vi "test - Clear CSM Queue.vi"(8 "error in (no error)":errorcluster, 11 "TestCase in":refnum<class "testcase-Basic-Function.lvclass">) -> (0 "error out":errorcluster, 3 "TestCase out":refnum<class "testcase-Basic-Function.lvclass">)   [LabVIEW 2017, in "testcase-Basic-Function.lvclass"]
uses:
  testcase-Basic-Function.lvclass
  src/user.lib/_NEVSTOP/Communicable State Machine(CSM)/_Support/CSMQ/_CSMOFGVOPER.ctl
  src/user.lib/_NEVSTOP/Communicable State Machine(CSM)/AdvanceAPI/CSM - Revert Arguments-Safe String.vi
  src/user.lib/_NEVSTOP/Communicable State Machine(CSM)/_Shared/Trim Single-line Text.vi
  src/user.lib/_NEVSTOP/Communicable State Machine(CSM)/AdvanceAPI/CSM - Make String Arguments Safe.vi
  src/user.lib/_NEVSTOP/Communicable State Machine(CSM)/AdvanceAPI/CSM - Break Down Multiple States String.vi
  src/user.lib/_NEVSTOP/Communicable State Machine(CSM)/AdvanceAPI/CSM - Compact Multiple States.vi
  src/user.lib/_NEVSTOP/Communicable State Machine(CSM)/AdvanceAPI/CSM - Keywords.vi
  <vilib>/addons/_JKI Toolkits/VI Tester/TestCase.llb/TestCase.lvclass
  src/user.lib/_NEVSTOP/Communicable State Machine(CSM)/Communicable State Machine.lvlib
  C:/Program Files (x86)/National Instruments/LabVIEW 2017/vi.lib/addons/_JKI Toolkits/VI Tester/TestCase.llb/TestCase.lvclass
panel:
  out "# pending insert":i32
  out "# pending remove":i32
  out "#Flushed":cluster{i32, i32}
  out "#elements in queue":i32
  out "error out 5":errorcluster
  out "error out 4":errorcluster
  out "error out 3":errorcluster
  out "error out 2":errorcluster
  out "error out 1":errorcluster
  out "State History":string
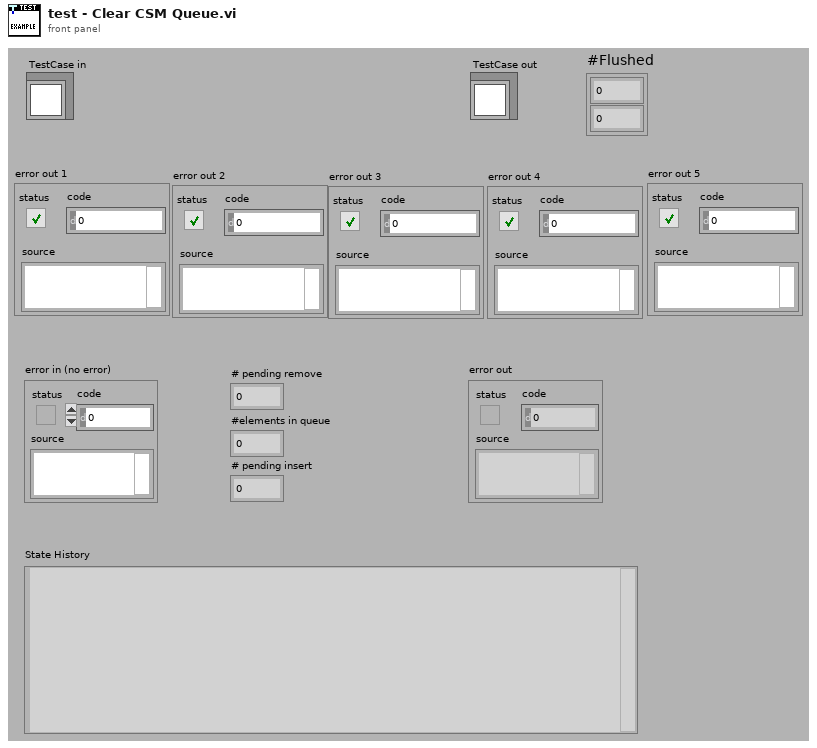
[diagram p1: front panel]
types:
  T1 = enum32{"Invalid", "Standard", "Closed", "Hidden", "Minimized", "Maximized"}
  T2 = enum32{"invalid app kind", "Development System", "Run Time System", "Student Edition", "Embedded LabVIEW", "Evaluation", "Custom"}
  T3 = typedef "Communicable State Machine.lvlib/_CSMOFGVOPER.ctl" = enum16{"Create If not Exist", "Get By Name", "List", "Check If Name Exists", "Release", "Module Status", "Create Status Event Handler", "Destroy Status Event Handler", "Clear Invalid Objs"}
  T4 = typedef "Communicable State Machine.lvlib/_CSM_Response Source Message.ctl" = cluster{"‘State":string, "’Arguments":string, "’Error":errorcluster}
  T5 = cluster{"Current VI Reference":refnum<vi>, "Close Panel on Exit?":bool}
  T6 = cluster{"Core":cluster{"Current VI Reference":refnum<vi>, "Close Panel on Exit?":bool}, "Your Boolean data":bool, "Your string data":string}
  T7 = typedef "Communicable State Machine.lvlib/_CSMObj.ctl" = cluster{"info":T8, "Refs":T10}
  T8 = typedef "Communicable State Machine.lvlib/_CSMObj-Info.ctl" = cluster{"Module Name":string, "Requested Name":string, "Group Name":string, "Mode":T9, "Allowed Messages":string[]}
  T9 = typedef "Communicable State Machine.lvlib/_CSM_MODE.ctl" = enum16{"Not Exist", "Stand Alone", "CSM", "Worker", "Worker Agent", "Chain Node", "Chain"}
  T10 = typedef "Communicable State Machine.lvlib/_CSMObj-Refs.ctl" = cluster{"WatchDogQ":refnum<queue>, "CSMDataDVR":refnum<data-value>, "Queue":T11, "GroupDataDVR":refnum<data-value>, "TagMap":refnum<data-value>, "ExitEvent":refnum<user-event>, "NewStateEvent":refnum<user-event>, "StatusEvent":refnum<user-event>, "InterruptEvent":refnum<user-event>}
  T11 = typedef "Communicable State Machine.lvlib/Priority Queue.ctl" = cluster{"HPriorityQ":refnum<queue>, "LowPriorityQ":refnum<queue>}
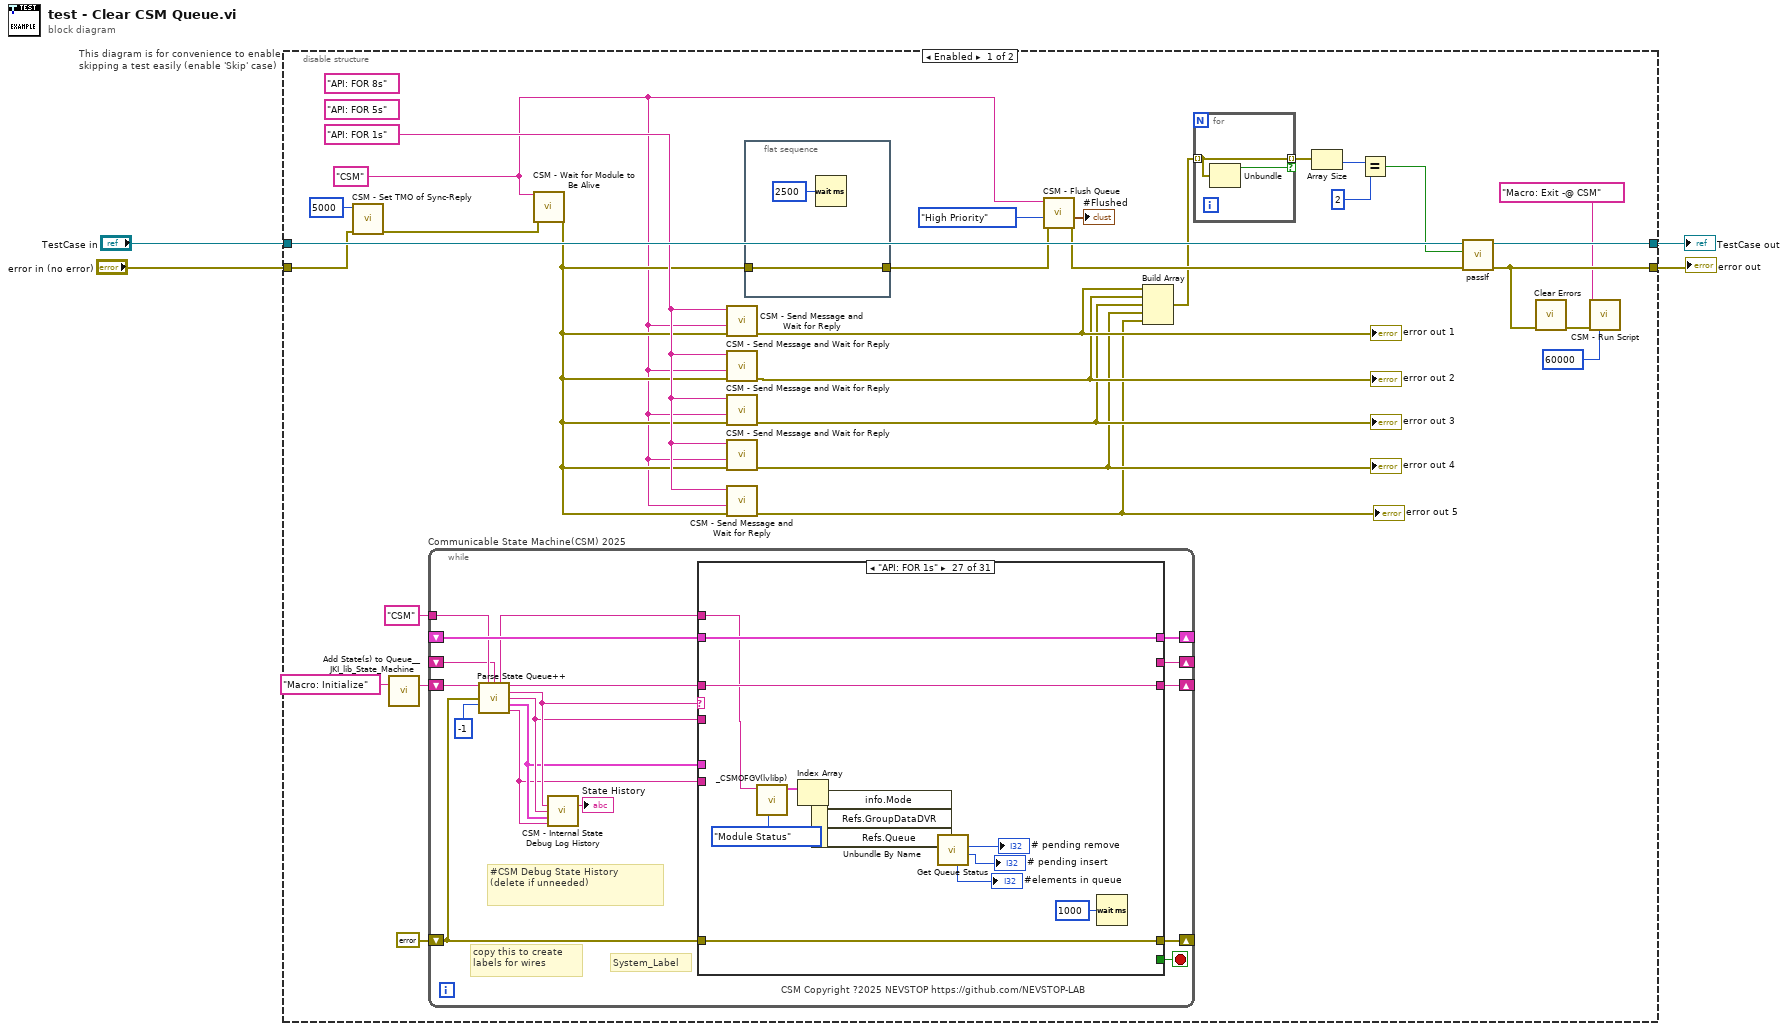
[diagram p0: block diagram]
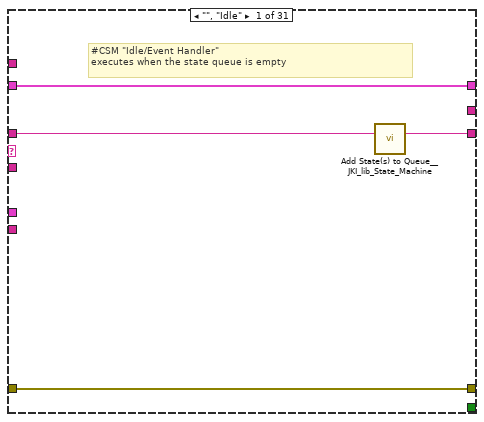
[diagram p2: hidden frame]
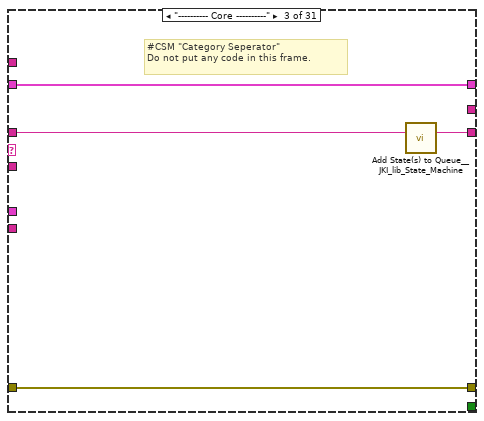
[diagram p4: hidden frame]
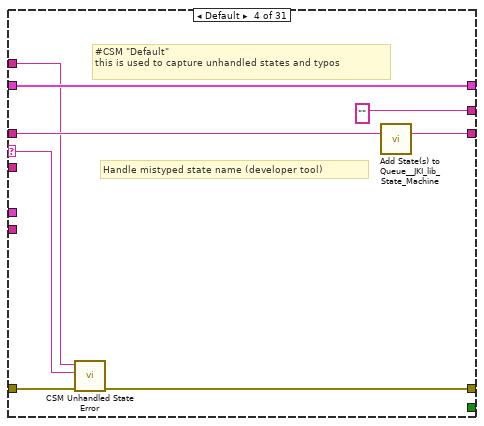
[diagram p5: hidden frame]
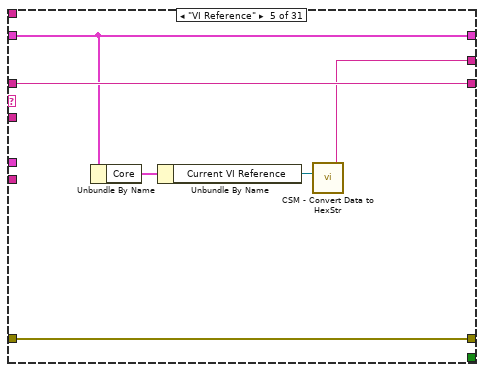
[diagram p6: hidden frame]
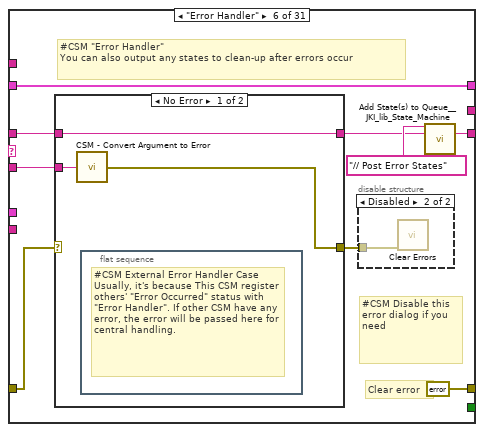
[diagram p7: hidden frame]
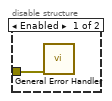
[diagram p8: hidden frame]
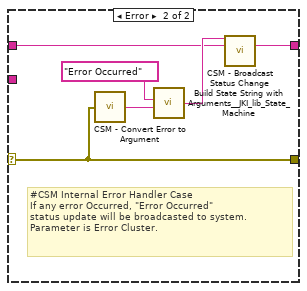
[diagram p9: hidden frame]
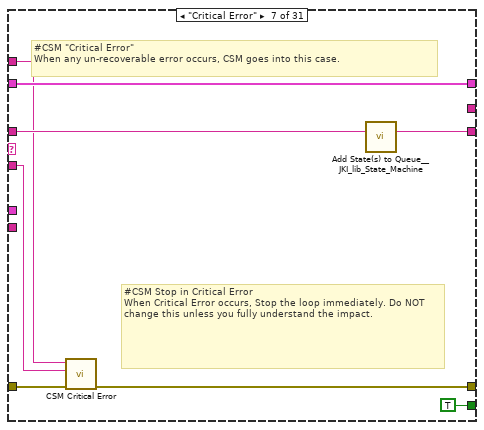
[diagram p10: hidden frame]
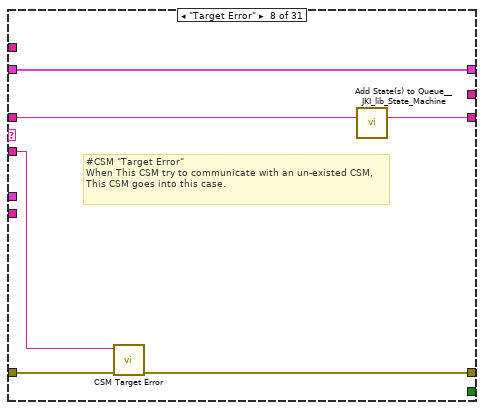
[diagram p11: hidden frame]
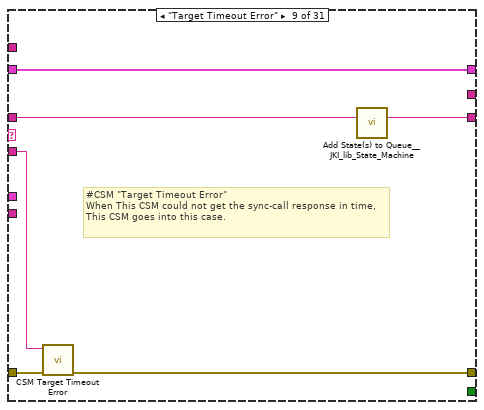
[diagram p12: hidden frame]
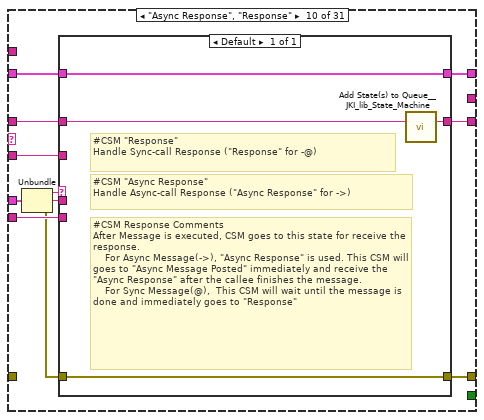
[diagram p13: hidden frame]
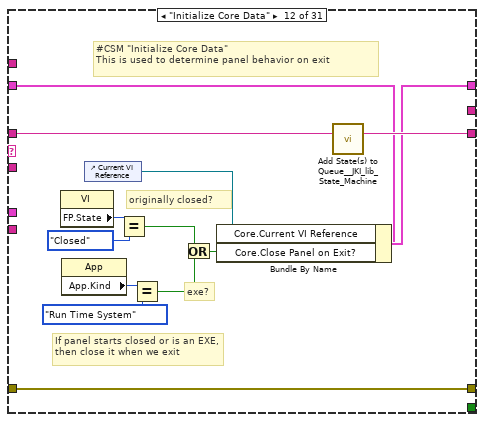
[diagram p15: hidden frame]
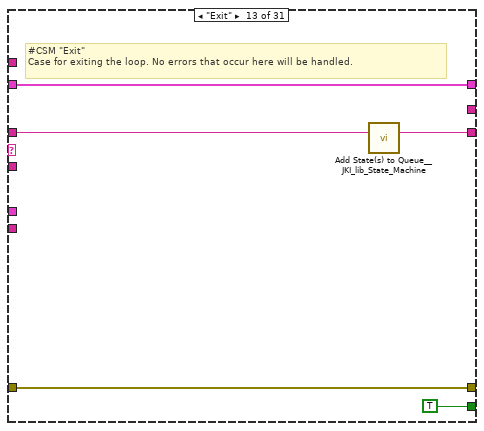
[diagram p16: hidden frame]
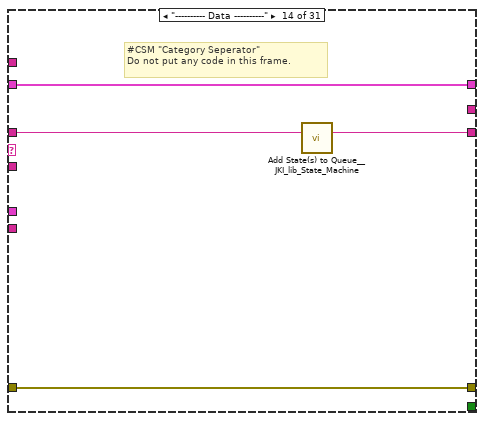
[diagram p17: hidden frame]
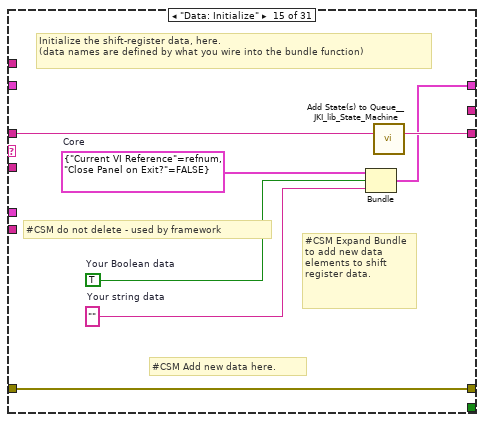
[diagram p18: hidden frame]
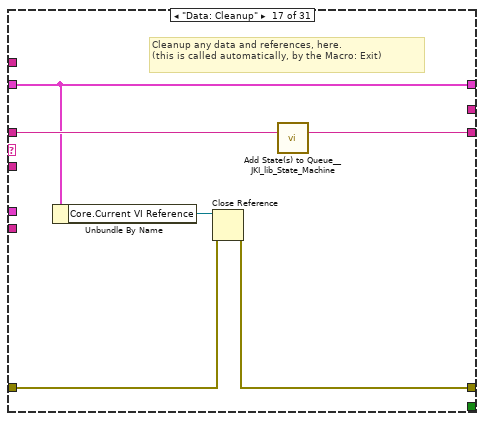
[diagram p20: hidden frame]
diagram:
  n1 = disable-structure "This diagram is for convenience to enable skipping a test easily (enable 'Skip' case)" shown="Enabled" {
    disable-tunnel: "TestCase in" -> [w26 w326]
    disable-tunnel: [w30 w324] -> w1
    disable-tunnel: [w29 w325] -> w3
    disable-tunnel: "error in (no error)" -> [w9 w323]
    frame Enabled {
      (unwired) "API: FOR 8s" ("State")
      (unwired) "API: FOR 5s" ("State")
      w25 = "API: FOR 1s" ("State")
      w21 = "CSM" ("Name (\"\" to Use UUID)")
      n2 = call "CSM - Set TMO of Sync-Reply.vi"("Error In"=w9, "TMO For Sync-Rep (ms) In"=5000 ("TMO for Sync-Rep(ms) In")) -> ("error out"=w8:errorcluster)  [unwired: 8 in, 1 out]
      n3 = call <vilib>:"Add State(s) to Queue__JKI_lib_State_Machine.vi"("State(s) in (\"\")"="Macro: Initialize" ("Init State(\"Macro: Initialize\")")) -> ("States Out"=w34:string)  [unwired: 14 in]
      n4 = while "Communicable State Machine(CSM) 2025" {
        shift-right: [w51] -> _
        shift-left: _ -> [w50]
        shift-right: [w54] -> _
        shift-left: errorcluster {"status"=FALSE, "code"=0, "source"=""} ("error out") -> [w49]
        shift-right: [w53] -> _
        shift-left: w34 -> [w55]
        tunnel: "CSM" ("Name (\"\" to Use UUID)") -> [w47]
        shift-right: [w48] -> _
        shift-left: _ -> [w41]
        stop <- w52 stop-if-true
        # "#CSM Debug State History\n(delete if unneeded)"
        # "copy this to create labels for wires"
        # "System_Label"
        # "CSM Copyright ?2025 NEVSTOP https://github.com/NEVSTOP-LAB"
        n5 = call "Parse State Queue++.vi"("State Queue"=w55, "Name (\"\" to Use UUID)"=w47, "Response Arguments"=w41, "Previous Error"=w49, "Dequeue (1 ms)"=-1 ("Timeout")) -> ("Name Used"=w42:string, "Remaining States"=w56:string, "Current State"=w46:string, "Arguments"=w45:string, "Additional Information"=w44:T4, "Source CSM"=w43:string)  [unwired: 5 in]
        n6 = call "CSM - Internal State Debug Log History.vi"("State"=w46, "Arguments (\"\")"=w45, ">> Response Source Message >>"=w44, "Source (\"\")"=w43) -> ("Debug Log"=→"State History":string)  [unwired: 11 in]
        n7 = case shown="\"API: FOR 1s\"" w46 {
          selector: w46 -> [_ _ _ w70 _ _ _ _ _ _ _ _ _ _ _ _ _ _ _ _ _ _ _ _ _ _ _ _ _ _ _]
          tunnel: w56 -> [w57 w62 w67 w74 w80 w86 w107 w113 w119 w127 w138 w152 w157 w161 w168 w170 w177 w181 w185 w191 w206 w275 w280 w287 w289 w293 w305 w309 w314 w318 w322]
          tunnel: w45 -> [_ _ _ _ _ w85 w103 w112 w117 w126 _ _ _ _ _ _ _ _ _ w186 w200 _ _ _ _ _ _ _ _ _ _]
          tunnel: w50 -> [w58 w61 w64 w72 w79 w89 w108 w114 w120 w129 w137 w145 w155 w158 _ w169 w172 w178 w183 w189 w202 w272 w277 w284 w288 w292 w304 w308 w311 w315 w319]
          tunnel: [w59 w63 w65 w68 w81 errorcluster {"status"=FALSE, "code"=0, "source"=""} ("error out") w104 w110 w116 w132 w139 w149 w154 w159 w165 w171 w173 w179 w182 w187 w203 w273 w278 w285 w290 w294 w306 w310 w312 w316 w320] -> w54
          tunnel: w49 -> [w59 w63 w65 w75 w81 w87 w109 w111 w118 _ w139 w149 w154 w159 w165 w171 w174 w179 w182 w188 w204 w273 w278 w285 w290 w294 w306 w310 w312 w316 w320]
          tunnel: [w60 w62 w66 w73 w80 w82 w106 w115 w121 w128 w138 w151 w156 w160 w167 w170 w176 w180 w184 w190 w205 w274 w279 w286 w289 w293 w305 w309 w313 w317 w321] -> w53
          tunnel: [_ _ _ _ _ _ TRUE _ _ _ _ _ TRUE _ _ _ _ _ _ _ _ _ _ _ _ _ _ _ _ _ _] -> w52
          tunnel: [w58 w61 w64 w72 w79 w89 w108 w114 w120 w130 w137 w150 w155 w158 w166 w169 w172 w178 w183 w189 w202 w272 w277 w284 w288 w292 w304 w308 w311 w315 w319] -> w51
          tunnel: w43 -> [_ _ _ _ _ _ _ _ _ w124 _ _ _ _ _ _ _ _ _ _ _ _ _ _ _ _ _ _ _ _ _]
          tunnel: w44 -> [_ _ _ _ _ _ _ _ _ w131 _ _ _ _ _ _ _ _ _ _ _ _ _ _ _ _ _ _ _ _ _]
          tunnel: [_ _ _ "" w76 _ _ _ _ _ _ _ _ _ _ _ _ _ _ _ _ _ _ _ _ _ _ _ _ _ _] -> w48
          tunnel: w42 -> [_ _ _ w69 _ _ w102 _ _ _ _ _ _ _ _ _ _ _ _ _ _ _ _ _ _ _ w301 _ _ _ _]
          frame "", "Idle" {
            # "#CSM \"Idle/Event Handler\"\nexecutes when the state queue is empty"
            n8 = call <vilib>:"Add State(s) to Queue__JKI_lib_State_Machine.vi"("State(s) in (\"\")"=w57) -> ("States Out"=w60:string)  [unwired: 14 in]
          }
          frame "CSM Documentation" {
            # "#CSM README FIRST\n\nCommunicable State Machine(CSM) is a LabVIEW application framework that builds upon JKI State Machine(JKISM). It follows the pattern of JKISM and extends the keywords to describe message communication between modules, including concepts such as Sync-Message, Async-Message, Subscription/Unsubscription of status - essential elements for creating reusable code modules. For more information, please visit the CSM wiki: https://nevstop-lab.github.io/CSM-Wiki/\n\nFor instructions on JKI State Machine, visit: http://jki.net/state-machine/\nFor information about CSM, visit: https://github.com/NEVSTOP-LAB"
            # "#CSM \"Documentation\"\nCase for holding CSM Documenation"
          }
          frame "---------- Core ----------" {
            # "#CSM \"Category Seperator\"\nDo not put any code in this frame."
            n9 = call <vilib>:"Add State(s) to Queue__JKI_lib_State_Machine.vi"("State(s) in (\"\")"=w67) -> ("States Out"=w66:string)  [unwired: 14 in]
          }
          frame Default {
            # "#CSM \"Default\"\nthis is used to capture unhandled states and typos"
            # "Handle mistyped state name (developer tool)"
            n10 = call "CSM Unhandled State Error.vi"("error in (no error)"=w75, "Undefined State"=w70, "CSM Name"=w69) -> ("error out"=w68:errorcluster)  [unwired: 8 in]
            n11 = call <vilib>:"Add State(s) to Queue__JKI_lib_State_Machine.vi"("State(s) in (\"\")"=w74) -> ("States Out"=w73:string)  [unwired: 14 in]
          }
          frame "VI Reference" {
            n12 = Unbundle By Name(w79) -> ("Core"=w78:T5)
            n13 = Unbundle By Name(w78) -> ("Current VI Reference"=w77:refnum<vi>)
            n14 = call "CSM - Convert Data to HexStr.vi"("Variant"=w77) -> ("HEX String (0-9,A-F)"=w76:string)  [unwired: 8 in]
          }
          frame "Error Handler" {
            # "#CSM Disable this error dialog if you need"
            # "#CSM \"Error Handler\"\nYou can also output any states to clean-up after errors occur"
            # "Clear error"
            n15 = case shown="No Error" w87 {
              selector: w87 -> [_ w96]
              tunnel: [w95 w98] -> w83
              tunnel: w86 -> [w95 w97]
              tunnel: w85 -> [w94 _]
              tunnel: [w93 w96] -> w88
              frame No Error {
                n16 = call "CSM - Convert Argument to Error.vi"("Argument"=w94) -> ("Error"=w93:errorcluster)  [unwired: 4 in]
                n17 = flat-sequence {
                  frame #0 {
                    # "#CSM External Error Handler Case\nUsually, it's because This CSM register others' \"Error Occurred\" status with \"Error Handler\". If other CSM have any error, the error will be passed here for central handling."
                  }
                }
              }
              frame Error {
                # "#CSM Internal Error Handler Case \nIf any error Occurred, \"Error Occurred\" \nstatus update will be broadcasted to system.\nParameter is Error Cluster."
                n18 = call "CSM - Convert Error to Argument.vi"("Error"=w96) -> ("Argument"=w100:string)  [unwired: 4 in]
                n19 = call <vilib>:"Build State String with Arguments__JKI_lib_State_Machine.vi"("Arguments (\"\")"=w100, "State"="Error Occurred" ("Status with Arguments")) -> ("State with Arguments"=w99:string)  [unwired: 4 in]
                n20 = call "CSM - Broadcast Status Change.vi"("Status With Arguments"=w99, "State Queue"=w97) -> ("Remaining States"=w98:string)  [unwired: 13 in]
              }
            }
            n21 = disable-structure shown="Disabled" {
              disable-tunnel: w88 -> [w91 w92]
              frame Enabled {
                n22 = call <vilib>:"General Error Handler.vi"("error in (no error)"=w91) -> ()  [unwired: 10 in, 5 out]
              }
              frame Disabled {
                n23 = call <vilib>:"Clear Errors.vi"("error in (no error)"=w92) -> ()  [unwired: 5 in, 2 out]
              }
            }
            n24 = call <vilib>:"Add State(s) to Queue__JKI_lib_State_Machine.vi"("State(s) in Front (\"\")"="// Post Error States", "State(s) in (\"\")"=w83) -> ("States Out"=w82:string)  [unwired: 13 in]
          }
          frame "Critical Error" {
            # "#CSM Stop in Critical Error\nWhen Critical Error occurs, Stop the loop immediately. Do NOT change this unless you fully understand the impact."
            # "#CSM \"Critical Error\"\nWhen any un-recoverable error occurs, CSM goes into this case."
            n25 = call "CSM Critical Error.vi"("error in (no error)"=w109, "Arugments (As Reason)"=w103, "CSM Name"=w102) -> ("error out"=w104:errorcluster)  [unwired: 8 in]
            n26 = call <vilib>:"Add State(s) to Queue__JKI_lib_State_Machine.vi"("State(s) in (\"\")"=w107) -> ("States Out"=w106:string)  [unwired: 14 in]
          }
          frame "Target Error" {
            # "#CSM \"Target Error\"\nWhen This CSM try to communicate with an un-existed CSM, This CSM goes into this case."
            n27 = call "CSM Target Error.vi"("error in (no error)"=w111, "Arguments (As CSM Name)"=w112) -> ("error out"=w110:errorcluster)  [unwired: 9 in]
            n28 = call <vilib>:"Add State(s) to Queue__JKI_lib_State_Machine.vi"("State(s) in (\"\")"=w113) -> ("States Out"=w115:string)  [unwired: 14 in]
          }
          frame "Target Timeout Error" {
            # "#CSM \"Target Timeout Error\"\nWhen This CSM could not get the sync-call response in time, This CSM goes into this case."
            n29 = call "CSM Target Timeout Error.vi"("error in (no error)"=w118, "Arguments (As CSM Name)"=w117) -> ("error out"=w116:errorcluster)  [unwired: 9 in]
            n30 = call <vilib>:"Add State(s) to Queue__JKI_lib_State_Machine.vi"("State(s) in (\"\")"=w119) -> ("States Out"=w121:string)  [unwired: 14 in]
          }
          frame "Async Response", "Response" {
            n31 = Unbundle(w131) -> ("‘State"=w125:string, "’Arguments"=w123:string, "’Error"=w122:errorcluster)
            n32 = case shown="Default" w125 {
              tunnel: [w136] -> w132
              tunnel: w122 -> [w136]
              tunnel: [w135] -> w130
              tunnel: w129 -> [w135]
              tunnel: [w133] -> w128
              tunnel: w127 -> [w134]
              tunnel: w126 -> [_]
              tunnel: w124 -> [_]
              tunnel: w123 -> [_]
              frame Default {
                # "#CSM Response Comments\nAfter Message is executed, CSM goes to this state for receive the response.\n    For Async Message(->), \"Async Response\" is used. This CSM will goes to \"Async Message Posted\" immediately and receive the \"Async Response\" after the callee finishes the message.\n    For Sync Message(@),  This CSM will wait until the message is done and immediately goes to \"Response\""
                # "#CSM \"Async Response\"\nHandle Async-call Response (\"Async Response\" for ->)"
                # "#CSM \"Response\"\nHandle Sync-call Response (\"Response\" for -@)"
                n33 = call <vilib>:"Add State(s) to Queue__JKI_lib_State_Machine.vi"("State(s) in (\"\")"=w134) -> ("States Out"=w133:string)  [unwired: 14 in]
              }
            }
          }
          frame "Async Message Posted" {
            # "#CSM \"Async Message Posted\"\nAfter Async Message is posted (-> or ->| ), CSM goes to this state for post-action.\nYou can use Argument - State to tell which Async Message is called."
          }
          frame "Initialize Core Data" {
            # "#CSM \"Initialize Core Data\"\nThis is used to determine panel behavior on exit"
            # "originally closed?"
            # "exe?"
            # "If panel starts closed or is an EXE, then close it when we exit"
            n34 = property class="VI"() -> ("FP.State"=w142:T1)  [unwired: 2 in, 2 out]
            n35 = property class="App"() -> ("App.Kind"=w148:T2)  [unwired: 2 in, 2 out]
            n36 = control-ref of="Current VI Reference"() -> (w143:refnum<vi>)
            n37 = Equal?(x=w142, y=T1."Closed" ("Front Panel Window:State")) -> (x = y?=w140:bool)
            n38 = Equal?(x=w148, y=T2."Run Time System" ("Application:Kind")) -> (x = y?=w146:bool)
            n39 = Or(x=w140, y=w146) -> (x .or. y?=w144:bool)
            n40 = Bundle By Name(cluster=w145, "Core.Current VI Reference"=w143, "Core.Close Panel on Exit?"=w144) -> (w150:T6)
            n41 = call <vilib>:"Add State(s) to Queue__JKI_lib_State_Machine.vi"("State(s) in (\"\")"=w152) -> ("States Out"=w151:string)  [unwired: 14 in]
          }
          frame "Exit" {
            # "#CSM \"Exit\"\nCase for exiting the loop. No errors that occur here will be handled."
            n42 = call <vilib>:"Add State(s) to Queue__JKI_lib_State_Machine.vi"("State(s) in (\"\")"=w157) -> ("States Out"=w156:string)  [unwired: 14 in]
          }
          frame "---------- Data ----------" {
            # "#CSM \"Category Seperator\"\nDo not put any code in this frame."
            n43 = call <vilib>:"Add State(s) to Queue__JKI_lib_State_Machine.vi"("State(s) in (\"\")"=w161) -> ("States Out"=w160:string)  [unwired: 14 in]
          }
          frame "Data: Initialize" {
            w162 = T5 {"Current VI Reference"=refnum, "Close Panel on Exit?"=FALSE}  # Core
            w164 = TRUE  # Your Boolean data
            w163 = ""  # Your string data
            # "#CSM do not delete - used by framework"
            # "#CSM Expand Bundle to add new data elements to shift register data."
            # "#CSM Add new data here."
            # "Initialize the shift-register data, here.\n(data names are defined by what you wire into the bundle function)"
            n44 = Bundle("Core"=w162, "Your Boolean data"=w164, "Your string data"=w163) -> (w166:T6)  [unwired: 1 in]
            n45 = call <vilib>:"Add State(s) to Queue__JKI_lib_State_Machine.vi"("State(s) in (\"\")"=w168) -> ("States Out"=w167:string)  [unwired: 14 in]
          }
          frame "Data: Update Indicators" {
          }
          frame "Data: Cleanup" {
            # "Cleanup any data and references, here.\n(this is called automatically, by the Macro: Exit)"
            n46 = Unbundle By Name(w172) -> ("Core.Current VI Reference"=w175:refnum<vi>)
            n47 = Close Reference(reference=w175, error in (no error)=w174) -> (error out=w173:errorcluster)
            n48 = call <vilib>:"Add State(s) to Queue__JKI_lib_State_Machine.vi"("State(s) in (\"\")"=w177) -> ("States Out"=w176:string)  [unwired: 14 in]
          }
          frame "---------- UI ----------" {
            # "#CSM \"Category Seperator\"\nDo not put any code in this frame."
            n49 = call <vilib>:"Add State(s) to Queue__JKI_lib_State_Machine.vi"("State(s) in (\"\")"=w181) -> ("States Out"=w180:string)  [unwired: 14 in]
          }
          frame "UI: Initialize" {
            # "#CSM \"UI: Initialize\"\nInitialize the User Interface, here.\n(this is called automatically, by the Macro: Init)"
            n50 = call <vilib>:"Add State(s) to Queue__JKI_lib_State_Machine.vi"("State(s) in (\"\")"=w185) -> ("States Out"=w184:string)  [unwired: 14 in]
          }
          frame "UI: Cursor Set" {
            # "#CSM \"UI: Cursor Set\"\nSet and Unset Cursor Busy.\n(Usage: \"UI: Cursor Set >> Busy|Idle\")"
            # "Argument"
            n51 = disable-structure shown="TARGET_TYPE!=Windows" {
              disable-tunnel: w188 -> [w194 w199]
              disable-tunnel: [w193 w199] -> w187
              disable-tunnel: w186 -> [w192 _]
              frame condition #0 (active) {
                n52 = case shown="\"Idle\", Default" w192 {
                  tunnel: w194 -> [w196 w198]
                  tunnel: [w195 w197] -> w193
                  frame "Idle", Default {
                    n53 = call <vilib>:"Unset Busy.vi"("error in (no error)"=w196) -> ("error out"=w195:errorcluster)  [unwired: 10 in]
                  }
                  frame "Busy" {
                    n54 = call <vilib>:"Set Busy.vi"("error in (no error)"=w198) -> ("error out"=w197:errorcluster)  [unwired: 9 in, 1 out]
                  }
                }
              }
              frame condition #1 {
              }
            }
            n55 = call <vilib>:"Add State(s) to Queue__JKI_lib_State_Machine.vi"("State(s) in (\"\")"=w191) -> ("States Out"=w190:string)  [unwired: 14 in]
          }
          frame "UI: Front Panel State" {
            # "#CSM \"UI: Front Panel State\"\nSet Front Panel Open or Closed\n(Usage: \"UI: Front Panel State >> Open|Close\")"
            # "Argument"
            n56 = Unbundle By Name(w202) -> ("Core.Current VI Reference"=w201:refnum<vi>)
            n57 = call <vilib>:"Add State(s) to Queue__JKI_lib_State_Machine.vi"("State(s) in (\"\")"=w206) -> ("States Out"=w205:string)  [unwired: 14 in]
            n58 = case shown="\"Close\", \"Closed\"" w200 {
              tunnel: w204 -> [w212 w227 w238 w251 w264]
              tunnel: [w214 w228 w240 w253 w266] -> w203
              tunnel: w201 -> [w213 w225 w239 w252 w265]
              frame "Open", "Standard", Default {
                w207 = T1."Standard" ("State")
                n59 = property class="VI"(reference=w213, error in=w212) -> (reference out=w210:refnum<vi>, error out=w211:errorcluster, "FP.State"=w209:T1)
                n60 = Not Equal?(x=w209, y=w207) -> (x != y?=w208:bool)
                n61 = case shown="True" w208 {
                  tunnel: [w218 w220] -> w214
                  tunnel: w211 -> [w217 w220]
                  tunnel: w210 -> [w216 _]
                  tunnel: w207 -> [w215 _]
                  frame True {
                    n62 = invoke class="VI" method="FP.Open"(reference=w216, error in=w217, "Activate"=TRUE, "State"=w215) -> (error out=w218:errorcluster)  [unwired: 1 in, 4 out]
                  }
                  frame False {
                  }
                }
              }
              frame "Close", "Closed" {
                n63 = property class="VI"(reference=w225, error in=w227) -> (reference out=w224:refnum<vi>, error out=w226:errorcluster, "FP.State"=w222:T1)
                n64 = Not Equal?(x=w222, y=T1."Closed" ("Front Panel Window:State")) -> (x != y?=w221:bool)
                n65 = case shown="False" w221 {
                  tunnel: [w229 w232] -> w228
                  tunnel: w226 -> [w229 w231]
                  tunnel: w224 -> [_ w230]
                  frame False {
                  }
                  frame True {
                    n66 = invoke class="VI" method="FP.Close"(reference=w230, error in=w231) -> (error out=w232:errorcluster)  [unwired: 1 in, 2 out]
                  }
                }
              }
              frame "Hidden", "Hide" {
                w233 = T1."Hidden" ("State")
                n67 = property class="VI"(reference=w239, error in=w238) -> (reference out=w236:refnum<vi>, error out=w237:errorcluster, "FP.State"=w235:T1)
                n68 = Not Equal?(x=w235, y=w233) -> (x != y?=w234:bool)
                n69 = case shown="True" w234 {
                  tunnel: [w244 w245] -> w240
                  tunnel: w237 -> [w243 w245]
                  tunnel: w236 -> [w242 _]
                  tunnel: w233 -> [w241 _]
                  frame True {
                    n70 = invoke class="VI" method="FP.Open"(reference=w242, error in=w243, "State"=w241) -> (error out=w244:errorcluster)  [unwired: 2 in, 4 out]
                  }
                  frame False {
                  }
                }
              }
              frame "Minimize", "Minimized" {
                w246 = T1."Minimized" ("State")
                n71 = property class="VI"(reference=w252, error in=w251) -> (reference out=w249:refnum<vi>, error out=w250:errorcluster, "FP.State"=w248:T1)
                n72 = Not Equal?(x=w248, y=w246) -> (x != y?=w247:bool)
                n73 = case shown="True" w247 {
                  tunnel: [w257 w258] -> w253
                  tunnel: w250 -> [w256 w258]
                  tunnel: w249 -> [w255 _]
                  tunnel: w246 -> [w254 _]
                  frame True {
                    n74 = invoke class="VI" method="FP.Open"(reference=w255, error in=w256, "State"=w254) -> (error out=w257:errorcluster)  [unwired: 2 in, 4 out]
                  }
                  frame False {
                  }
                }
              }
              frame "Maximize", "Maximized" {
                w259 = T1."Maximized" ("State")
                n75 = property class="VI"(reference=w265, error in=w264) -> (reference out=w262:refnum<vi>, error out=w263:errorcluster, "FP.State"=w261:T1)
                n76 = Not Equal?(x=w261, y=w259) -> (x != y?=w260:bool)
                n77 = case shown="True" w260 {
                  tunnel: [w270 w271] -> w266
                  tunnel: w263 -> [w269 w271]
                  tunnel: w262 -> [w268 _]
                  tunnel: w259 -> [w267 _]
                  frame True {
                    n78 = invoke class="VI" method="FP.Open"(reference=w268, error in=w269, "State"=w267) -> (error out=w270:errorcluster)  [unwired: 2 in, 4 out]
                  }
                  frame False {
                  }
                }
              }
            }
          }
          frame "---------- Macro ----------" {
            # "#CSM \"Category Seperator\"\nDo not put any code in this frame."
            n79 = call <vilib>:"Add State(s) to Queue__JKI_lib_State_Machine.vi"("State(s) in (\"\")"=w275) -> ("States Out"=w274:string)  [unwired: 14 in]
          }
          frame "Macro: Initialize" {
            # "#CSM \"Macro: Initialize\"\nInitialization Macro (This is called once, when the VI starts)"
            n80 = call <vilib>:"Add State(s) to Queue__JKI_lib_State_Machine.vi"("State(s) in Front (\"\")"="Data: Initialize\nInitialize Core Data\nData: Update Indicators", "State(s) in (\"\")"=w280) -> ("States Out"=w279:string)  [unwired: 13 in]
          }
          frame "Macro: Exit" {
            # "#CSM \"Macro: Exit\"\nExit Macro (This is called once, when the VI exits)"
            n81 = call <vilib>:"Add State(s) to Queue__JKI_lib_State_Machine.vi"("State(s) in Front (\"\")"="//Exit Sub-Modules ", "State(s) at Back (\"\")"="Data: Cleanup\nExit") -> ("States Out"=w282:string)  [unwired: 13 in]
            n82 = call <vilib>:"Add State(s) to Queue__JKI_lib_State_Machine.vi"("State(s) in Front (\"\")"=w282, "State(s) in (\"\")"=w287) -> ("States Out"=w286:string)  [unwired: 13 in]
          }
          frame "---------- API ----------" {
            # "#CSM \"Category Seperator\"\nDo not put any code in this frame."
          }
          frame "API: FOR 5s" {
            n83 = Wait (ms)(milliseconds to wait=u32 5000) -> ()  [unwired: 1 out]
          }
          frame "API: FOR 1s" {
            n84 = call "_CSMOFGV(lvlibp).vi"("Operation"=_CSMOFGVOPER."Module Status", "Name (\"\" to Use UUID) In"=w301) -> ("Array"=w299:T7[])  [unwired: 7 in, 2 out]
            n85 = Index Array(array=w299) -> (element=w300:T7)  [unwired: 1 in]
            n86 = Unbundle By Name(w300) -> ("Refs.Queue"=w298:T11)  [unwired: 2 out]
            n87 = call "Get Queue Status.vi"("Priority Queue In"=w298) -> ("# Pending Insert"=→"# pending insert":i32, "# Pending Remove"=→"# pending remove":i32, "# Elements In Queue"=→"#elements in queue":i32)  [unwired: 6 in, 2 out]
            n88 = Wait (ms)(milliseconds to wait=u32 1000) -> ()  [unwired: 1 out]
          }
          frame "API: FOR 8s" {
            n89 = Wait (ms)(milliseconds to wait=u32 8000) -> ()  [unwired: 1 out]
          }
          frame "---------- Action ----------" {
            # "#CSM \"Category Seperator\"\nDo not put any code in this frame."
            n90 = call <vilib>:"Add State(s) to Queue__JKI_lib_State_Machine.vi"("State(s) in (\"\")"=w314) -> ("States Out"=w313:string)  [unwired: 14 in]
          }
          frame "Action: action1" {
            # "#CSM \"Internal State\"\nThis category is used for holding internal states"
            n91 = call <vilib>:"Add State(s) to Queue__JKI_lib_State_Machine.vi"("State(s) in (\"\")"=w318) -> ("States Out"=w317:string)  [unwired: 14 in]
          }
          frame "Action: action2" {
            # "#CSM \"Internal State\"\nThis category is used for holding internal states"
            n92 = call <vilib>:"Add State(s) to Queue__JKI_lib_State_Machine.vi"("State(s) in (\"\")"=w322) -> ("States Out"=w321:string)  [unwired: 14 in]
          }
        }
      }
      n93 = call "CSM - Wait for Module to Be Alive.vi"("CSM Name"=w21, "error in (no error)"=w8) -> ("error out"=w23:errorcluster)  [unwired: 11 in, 2 out]
      n94 = call "CSM - Send Message and Wait for Reply.vi"("Error In (No Error)"=w23, "Target Module"=w21, "State"=w25) -> ("error out"=w19:errorcluster)  [unwired: 6 in, 2 out]
      "error out 1" <- w19
      n95 = call "CSM - Send Message and Wait for Reply.vi"("Error In (No Error)"=w23, "Target Module"=w21, "State"=w25) -> ("error out"=w18:errorcluster)  [unwired: 6 in, 2 out]
      "error out 2" <- w18
      n96 = call "CSM - Send Message and Wait for Reply.vi"("Error In (No Error)"=w23, "Target Module"=w21, "State"=w25) -> ("error out"=w17:errorcluster)  [unwired: 6 in, 2 out]
      "error out 3" <- w17
      n97 = call "CSM - Send Message and Wait for Reply.vi"("Error In (No Error)"=w23, "Target Module"=w21, "State"=w25) -> ("error out"=w16:errorcluster)  [unwired: 6 in, 2 out]
      "error out 4" <- w16
      n98 = call "CSM - Send Message and Wait for Reply.vi"("Error In (No Error)"=w23, "Target Module"=w21, "State"=w25) -> ("error out"=w15:errorcluster)  [unwired: 6 in, 2 out]
      "error out 5" <- w15
      n99 = flat-sequence {
        tunnel: [w37] -> w24
        tunnel: w23 -> [w37]
        frame #0 {
          n100 = Wait (ms)(milliseconds to wait=u32 2500) -> ()  [unwired: 1 out]
        }
      }
      n101 = call "CSM - Flush Queue.vi"("Error In"=w24, "Option (Low Priority As Default)"=enum16{"All", "High Priority", "Low Priority"}."High Priority" ("Option(Low Priority as Default)"), "CSM Name"=w21) -> ("error out"=w22:errorcluster, "#Flushed"=→"#Flushed":cluster{i32, i32})  [unwired: 6 in, 1 out]
      n102 = Build Array(w19, w18, w17, w16, w15) -> (w14:errorcluster[])
      n103 = for {
        tunnel: w14 -> [w36] mode=indexing
        tunnel: [w36] -> w13 mode=indexing if=w35
        n104 = Unbundle(w36) -> ("status"=w35:bool)  [unwired: 2 out]
      }
      n105 = Array Size(array=w13) -> (size(s)=w12:i32)
      n106 = Equal?(x=w12, y=2) -> (x = y?=w10:bool)
      n107 = call-dynamic "passIf.vi"("error in (no error)"=w22, "pass"=w10, "TestCase in"=w26) -> ("error out"=w29:errorcluster, "TestCase out"=w30:refnum<class "testcase-Basic-Function.lvclass">)  [unwired: 7 in]
      n108 = call <vilib>:"Clear Errors.vi"("error in (no error)"=w29) -> ("error out"=w28:errorcluster)  [unwired: 5 in, 1 out]
      n109 = call "CSM - Run Script.vi"("CSM Scripts"="Macro: Exit -@ CSM", "error in (no error)"=w28, "Response Timeout (-2 Using Global Settings)"=60000) -> ()  [unwired: 10 in, 3 out]
    }
    frame Disabled {
      # "skip test result while test is under development"
      n110 = call <vilib>:"skip.vi"("error in (no error)"=w323, "TestCase in"=w326) -> ("error out"=w325:errorcluster, "TestCase out"=w324:refnum<class "testcase-Basic-Function.lvclass">)  [unwired: 8 in]
    }
  }
  "error out" <- w3
  "TestCase out" <- w1
